vi "Zadatak1_NILI.vi"() -> ()   [LabVIEW 2013]
panel:
  out "Boolean":bool
  in  "C":bool
  in  "B":bool
  in  "A":bool
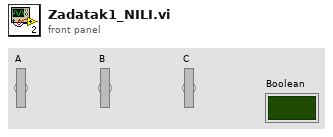
[diagram p1: front panel]
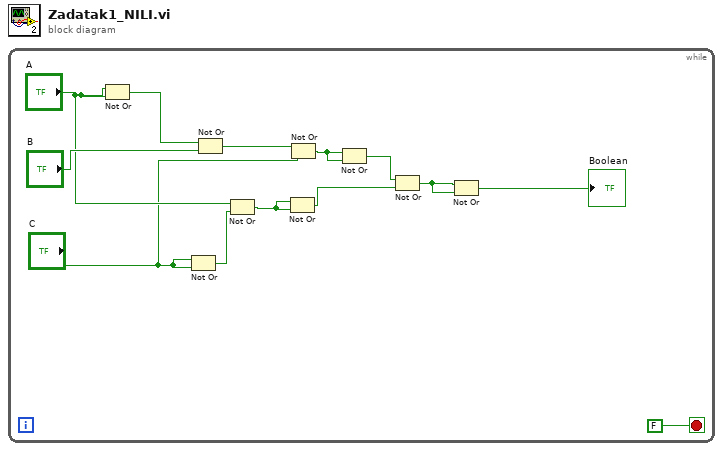
[diagram p0: block diagram]
diagram:
  n1 = while {
    stop <- FALSE stop-if-true
    n2 = Not Or(1:"A", 2:"A") -> (0:w11:bool)
    n3 = Not Or(1:"C", 2:"C") -> (0:w9:bool)
    n4 = Not Or(1:"B", 2:w11) -> (0:w7:bool)
    n5 = Not Or(1:w9, 2:"A") -> (0:w8:bool)
    n6 = Not Or(1:w8, 2:w8) -> (0:w3:bool)
    n7 = Not Or(1:"C", 2:w7) -> (0:w5:bool)
    n8 = Not Or(1:w5, 2:w5) -> (0:w4:bool)
    n9 = Not Or(1:w3, 2:w4) -> (0:w2:bool)
    n10 = Not Or(1:w2, 2:w2) -> (0:→"Boolean":bool)
  }
